vi "Transport.vi"(4 "Async Elements":refnum<class "Async Elements.lvclass">, 6 "VI Ref":refnum<vi>, 7 "Actor in":refnum<class "Actor.lvclass">, 10 "Refs":refnum<class "Refs.lvclass">) -> (0 "Error out":errorcluster, 5 "Actor out":refnum<class "Actor.lvclass">)   [LabVIEW 2020, in "jettl.lvlib" / "Queue Transport.lvlib"]
uses:
  Queue Transport.lvlib
  Actor/Actor.lvclass
  Refs/Refs.lvclass
  Async Elements/Async Elements.lvclass
  Base Async Elements/Base Async Elements/Base Async Elements.lvclass/Base Async Elements.ctl
  Base Attributes/Base Attributes/Base Attributes.lvclass/Base Attributes.ctl
  Queue Transport/Queue Transport.lvclass/Queue Transport.ctl
  Read Address.vi
  Update Attributes A.vi
  Update Attributes B.vi
  Base Async Elements/Read Async Elements.vi
  Queue Transport/Read Address.vi
  Base Attributes/Init Attributes.vi
  Base Async Elements/Base Async Elements/Read Async Elements.vi
  Base Attributes/Base Attributes/Init Attributes.vi
  Queue Transport/Queue Transport.lvclass
  C:/git/jettl/src/jettl/jettl/Transport/Transport.lvclass
  Base Attributes/Base Attributes/Base Attributes.lvclass
  C:/git/jettl/src/jettl/jettl/Attributes/Attributes.lvclass
  Call.vi
  Stop jettl Msg/Stop/Stop.vi
  Stop jettl Msg/Stop/Call.vi
  Attributes/Attributes.lvclass
  Base Async Elements/Base Async Elements/Base Async Elements.lvclass
  Msg/Msg.lvclass
  Transport/Transport.lvclass
  Msg Output/Msg Output.lvclass
  jettl.lvlib
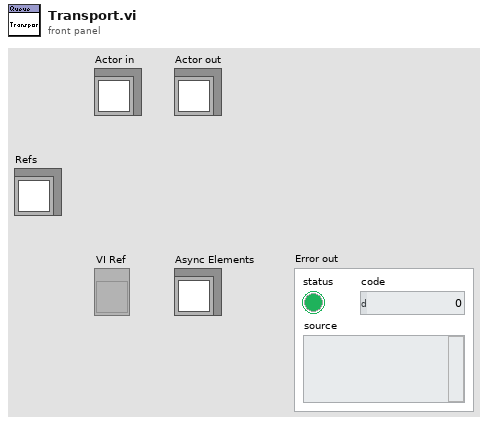
[diagram p1: front panel]
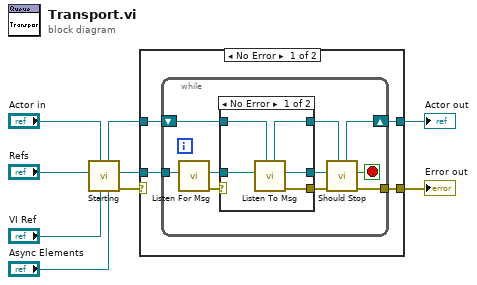
[diagram p0: block diagram]
diagram:
  n1 = call "Starting.vi"("Async Elements"="Async Elements", "VI Ref"="VI Ref", "Actor in"="Actor in", "Refs"="Refs") -> ("Error out"=w5:errorcluster, "Address"=w2:refnum<data-value>, "Actor out"=w7:refnum<class "Actor.lvclass">)  [unwired: 5 in]
  n2 = case shown="No Error" w5 {
    selector: w5 -> [_ w32]
    tunnel: [w10 w31] -> w8
    tunnel: [w13 w32] -> w9
    tunnel: w7 -> [w12 w31]
    tunnel: w2 -> [w11 _]
    frame No Error {
      n3 = while {
        shift-right: [w21] -> w10
        shift-left: w12 -> [w19]
        tunnel: [w22] -> w13
        tunnel: w11 -> [w17]
        stop <- w20 stop-if-true
        n4 = call "Listen For Msg.vi"("Address"=w17) -> ("Error out"=w15:errorcluster, "Msg"=w16:refnum<class "Msg.lvclass">)  [unwired: 9 in]
        n5 = case shown="No Error" w15 {
          selector: w15 -> [_ w29]
          tunnel: [w25 w29] -> w23
          tunnel: w19 -> [w28 w30]
          tunnel: [w26 w30] -> w18
          tunnel: w16 -> [w27 _]
          tunnel: [w24 _] -> w14
          frame No Error {
            n6 = call "Listen To Msg.vi"("Actor in"=w28, "Msg"=w27) -> ("Error out"=w25:errorcluster, "Msg Output"=w24:refnum<class "Msg Output.lvclass">, "Actor out"=w26:refnum<class "Actor.lvclass">)  [unwired: 7 in]
          }
          frame Error {
          }
        }
        n7 = call "Should Stop.vi"("Actor in"=w18, "Error in"=w23, "Msg Output"=w14) -> ("Error out"=w22:errorcluster, "Stop"=w20:bool, "Actor out"=w21:refnum<class "Actor.lvclass">)  [unwired: 6 in]
      }
    }
    frame Error {
    }
  }
  "Error out" <- w9
  "Actor out" <- w8
